vi "Main Page.vi"(8 "error in":errorcluster, 11 "Node Ptr":T2 format="%.0x") -> (0 "error out":errorcluster)   [LabVIEW 2020, in "Ballard ARINC 429 System Explorer.lvlib" / "Implementation.lvlib"]
uses:
  Implementation.lvlib
  <vilib>/NI VeriStand/Custom Device API/Custom Device API.lvlib
  Scripting/Ballard/Ballard ARINC 429 Scripting.lvlib
  Scripting/Ballard/Constants.vi
  <vilib>/NI VeriStand/Custom Device API/Custom Device Item Ref.ctl
  Shared/Initialization Method.ctl
panel:
  in  "Async Rx Execution":bool
  in  "General Header":cluster{"Section Name":string}={"Section Name"="Ballard ARINC 429 - Main"}
  in  "Initialization Method":T1
  in  "Core Number":i32=1 format="%o"
  in  "Number":i32=1 caption="PXI Slot Number"
  in  "SHDocVw.IWebBrowser":refnum<k7>(container)
  in  "Description":string
  in  "Name":string
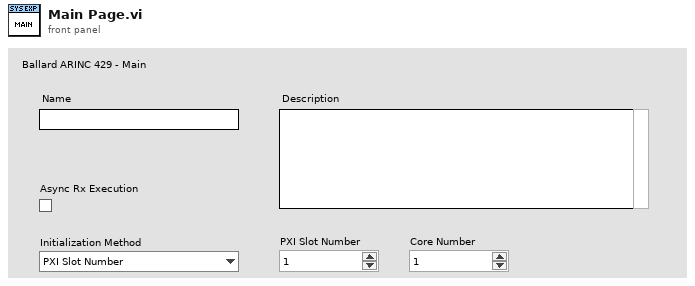
[diagram p1: front panel]
types:
  T1 = typedef "Initialization Method.ctl" = enum16{"PXI Slot Number", "Card Number", "Core Serial Number"}
  T2 = typedef "Custom Device API.lvlib/Custom Device Item Ref.ctl" = u64
  T3 = typedef "Device Parameters.ctl" = cluster{"initialization method":T1, "card number":i32, "PXI slot number":i32, "core number":i32, "core serial number":i32}
  T4 = typedef "Custom Device API.lvlib/Custom Device Item Info.ctl" = cluster{"Name":string, "Is Channel":bool, "GUID":string, "Is Waveform":bool}
  T5 = typedef "Custom Device API.lvlib/Custom Device Commands.ctl" = enum16{"Default", "Item renamed", "Shutdown", "Dynamic button pressed"}
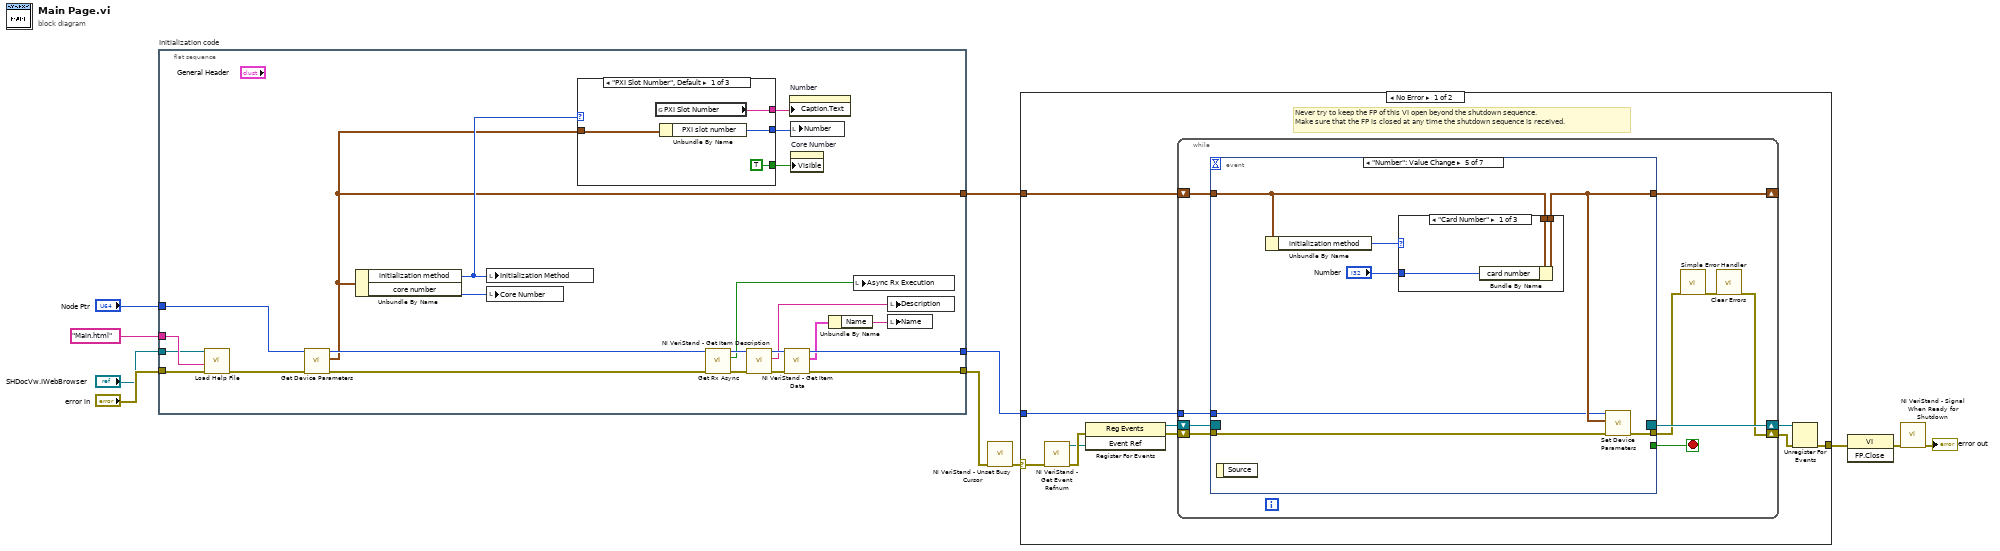
[diagram p0: block diagram]
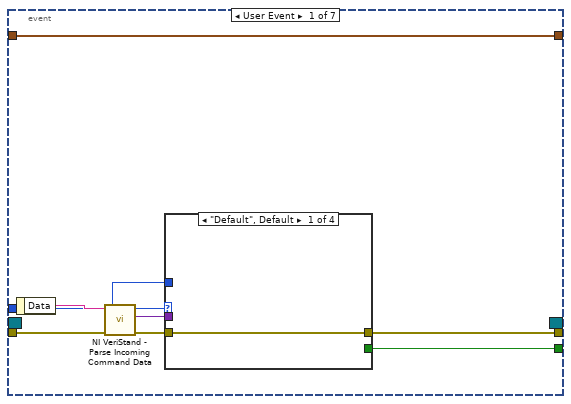
[diagram p2: hidden frame]
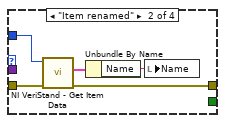
[diagram p3: hidden frame]
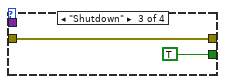
[diagram p4: hidden frame]
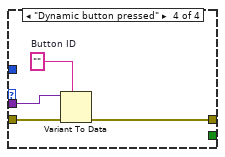
[diagram p5: hidden frame]
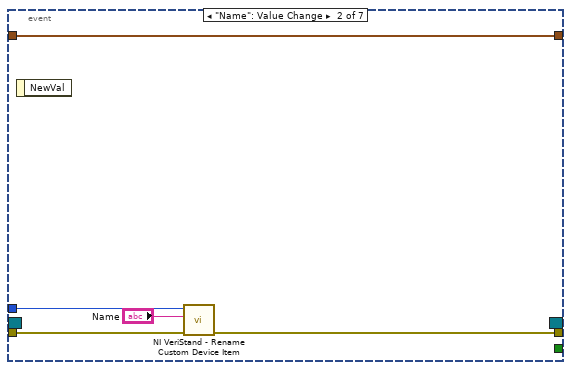
[diagram p6: hidden frame]
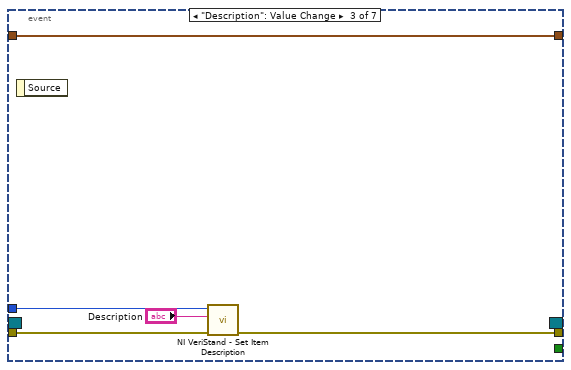
[diagram p7: hidden frame]
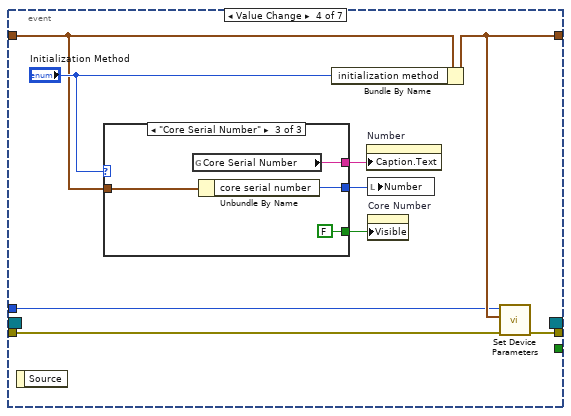
[diagram p8: hidden frame]
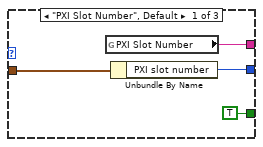
[diagram p9: hidden frame]
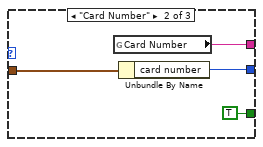
[diagram p10: hidden frame]
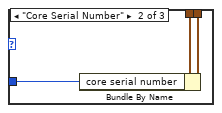
[diagram p11: hidden frame]
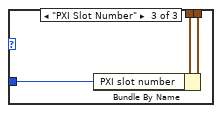
[diagram p12: hidden frame]
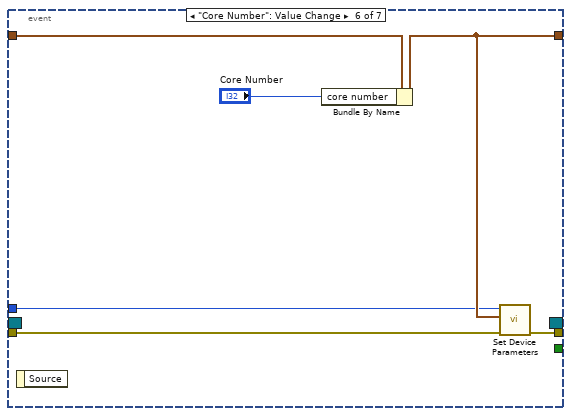
[diagram p13: hidden frame]
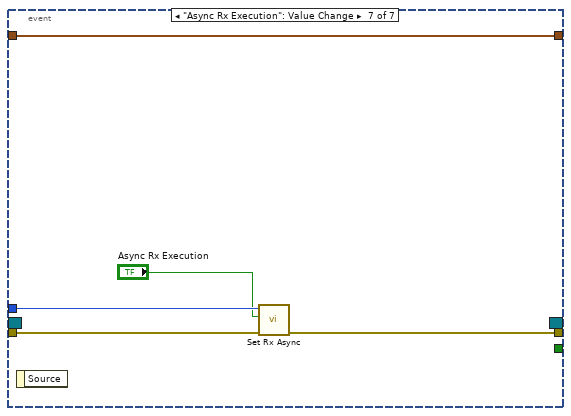
[diagram p14: hidden frame]
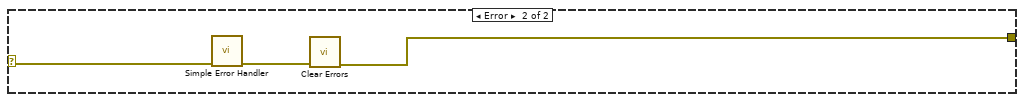
[diagram p15: hidden frame]
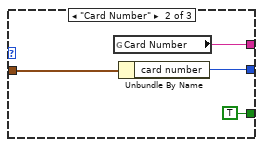
[diagram p16: hidden frame]
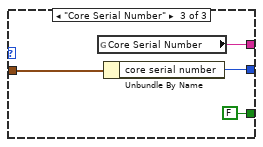
[diagram p17: hidden frame]
diagram:
  n1 = flat-sequence "Initialization code" {
    tunnel: "error in" -> [w27]
    tunnel: "Node Ptr" -> [w22]
    tunnel: [w30] -> w7
    tunnel: [w34] -> w4
    tunnel: "SHDocVw.IWebBrowser" -> [w25]
    tunnel: "Main.html" ("HTML File") -> [w26]
    tunnel: [w14] -> w1
    frame #0 {
      n2 = call "Load Help File.vi"("error in (no error)"=w27, "HTML File to Load"=w26, "Browser"=w25) -> ("error out"=w24:errorcluster)  [unwired: 8 in]
      n3 = call "Get Device Parameters.vi"("error in"=w24, "Ballard ARINC 429 custom device in"=w22) -> ("error out"=w18:errorcluster, "device parameters"=w14:T3, "Ballard ARINC 429 custom device out"=w23:T2)  [unwired: 7 in]
      n4 = Unbundle By Name(w14) -> ("initialization method"=w16:T1, "core number"=w21:i32)
      n5 = local write "Initialization Method"(w16) -> ()
      n6 = local write "Core Number"(w21) -> ()
      n7 = case shown="\"PXI Slot Number\", Default" w16 {
        tunnel: [w38 w42 w46] -> w15
        tunnel: w14 -> [w37 w41 w45]
        tunnel: [w36 w40 w44] -> w13
        tunnel: [TRUE ("Visible") TRUE ("Visible") FALSE ("Visible")] -> w12
        frame "PXI Slot Number", Default {
          n8 = global read "Constants.vi" "PXI Slot Number"() -> (w38:string)
          n9 = Unbundle By Name(w37) -> ("PXI slot number"=w36:i32)
        }
        frame "Card Number" {
          n10 = global read "Constants.vi" "Card Number"() -> (w42:string)
          n11 = Unbundle By Name(w41) -> ("card number"=w40:i32)
        }
        frame "Core Serial Number" {
          n12 = global read "Constants.vi" "Core Serial Number"() -> (w46:string)
          n13 = Unbundle By Name(w45) -> ("core serial number"=w44:i32)
        }
      }
      n14 = call "Get Rx Async.vi"("error in"=w18, "Ballard ARINC 429 custom device in"=w23) -> ("error out"=w19:errorcluster, "rx async?"=w17:bool, "Ballard ARINC 429 custom device out"=w20:T2)  [unwired: 7 in]
      n15 = call <vilib>:"NI VeriStand - Get Item Description.vi"("error in (no error)"=w19, "Item Ref in"=w20) -> ("error out"=w32:errorcluster, "Description"=w28:string, "Item Ref out"=w33:T2)  [unwired: 7 out]
      n16 = call <vilib>:"NI VeriStand - Get Item Data.vi"("error in (no error)"=w32, "Item Ref in"=w33) -> ("error out"=w30:errorcluster, "Item Info"=w31:T4, "Item Ref out"=w34:T2)  [unwired: 7 out]
      n17 = property on="Number" class="DigNum (strict)"("Caption.Text"=w15) -> ()  [unwired: 2 in, 2 out]
      n18 = local write "Number"(w13) -> ()
      n19 = property on="Core Number" class="DigNum (strict)"("Visible"=w12) -> ()  [unwired: 2 in, 2 out]
      n20 = Unbundle By Name(w31) -> ("Name"=w29:string)
      n21 = local write "Async Rx Execution"(w17) -> ()
      n22 = local write "Description"(w28) -> ()
      n23 = local write "Name"(w29) -> ()
    }
  }
  n24 = call <vilib>:"NI VeriStand - Unset Busy Cursor.vi"("error in (no error)"=w7) -> ("error out"=w6:errorcluster)  [unwired: 10 out]
  n25 = case shown="No Error" w6 {
    selector: w6 -> [w48 w148]
    tunnel: [w53 w146] -> w11
    tunnel: w4 -> [w49 _]
    tunnel: w1 -> [w47 _]
    frame No Error {
      # "Never try to keep the FP of this VI open beyond the shutdown sequence.\nMake sure that the FP is closed at any time the shutdown sequence is received."
      n26 = call <vilib>:"NI VeriStand - Get Event Refnum.vi"("error in (no error)"=w48) -> ("error out"=w56:errorcluster, "Event Ref"=w52:refnum<user-event>)  [unwired: 9 out]
      n27 = register-events(error in=w56, w52) -> (reference out=w50:refnum<event-registration>, error out=w51:errorcluster)  [unwired: 1 in]
      n28 = while {
        tunnel: w49 -> [w62]
        shift-right: [w59] -> w54
        shift-left: w51 -> [w65]
        shift-right: [w66] -> w55
        shift-left: w50 -> [w64]
        shift-right: [w57] -> _
        shift-left: w47 -> [w58]
        stop <- w63 stop-if-true
        n29 = event shown="[4] \"Number\": Value Change" {
          selector: w64 -> [_ _ _ _ _ _ _]
          dyn-events: [_ _ _ _ _ _ _] -> w66
          timeout: _ -> [_ _ _ _ _ _ _]
          tunnel: w65 -> [w75 w92 w96 w105 w123 w138 w144]
          tunnel: [w71 _ _ _ _ _ _] -> w63
          tunnel: [w70 w91 w95 w104 w122 w137 w141] -> w61
          tunnel: w62 -> [w69 w90 w97 w103 w120 w135 w143]
          tunnel: w58 -> [w67 w88 w93 w98 w125 w140 w145]
          tunnel: [w67 w88 w93 w106 w124 w139 w145] -> w57
          event User Event {
            n30 = event-data() -> ("Data"=w74:string)  [unwired: 1 out]
            n31 = call <vilib>:"NI VeriStand - Parse Incoming Command Data.vi"("error in (no error)"=w75, "Incoming data"=w74) -> ("error out"=w73:errorcluster, "Outgoing data"=w68:variant, "Action"=w72:T5)  [unwired: 7 out]
            n32 = case shown="\"Default\", Default" w72 {
              tunnel: w73 -> [w76 w81 w82 w87]
              tunnel: [_ _ TRUE _] -> w71
              tunnel: [w76 w78 w82 w84] -> w70
              tunnel: w69 -> [_ w80 _ _]
              tunnel: w68 -> [_ _ _ w86]
              frame "Default", Default {
              }
              frame "Item renamed" {
                n33 = call <vilib>:"NI VeriStand - Get Item Data.vi"("error in (no error)"=w81, "Item Ref in"=w80) -> ("error out"=w78:errorcluster, "Item Info"=w79:T4)  [unwired: 8 out]
                n34 = Unbundle By Name(w79) -> ("Name"=w77:string)
                n35 = local write "Name"(w77) -> ()
              }
              frame "Shutdown" {
              }
              frame "Dynamic button pressed" {
                w85 = ""  # Button ID
                n36 = Variant To Data(error in=w87, type=w85, Variant=w86) -> (error out=w84:errorcluster)  [unwired: 1 out]
              }
            }
          }
          event "Name": Value Change {
            n37 = event-data() -> ()  [unwired: 2 out]
            n38 = call <vilib>:"NI VeriStand - Rename Custom Device Item.vi"("error in (no error)"=w92, "New Name"="Name", "Item Ref in"=w90) -> ("error out"=w91:errorcluster)  [unwired: 1 in, 7 out]
          }
          event "Description": Value Change {
            n39 = event-data() -> ()  [unwired: 2 out]
            n40 = call <vilib>:"NI VeriStand - Set Item Description.vi"("error in (no error)"=w96, "Description"="Description", "Item Ref in"=w97) -> ("error out"=w95:errorcluster)  [unwired: 8 out]
          }
          event Value Change {
            n41 = event-data() -> ()  [unwired: 2 out]
            n42 = case shown="\"Core Serial Number\"" "Initialization Method" {
              tunnel: [w110 w114 w118] -> w102
              tunnel: w98 -> [w109 w113 w117]
              tunnel: [w108 w112 w116] -> w101
              tunnel: [TRUE ("Visible") TRUE ("Visible") FALSE ("Visible")] -> w100
              frame "PXI Slot Number", Default {
                n43 = global read "Constants.vi" "PXI Slot Number"() -> (w110:string)
                n44 = Unbundle By Name(w109) -> ("PXI slot number"=w108:i32)
              }
              frame "Card Number" {
                n45 = global read "Constants.vi" "Card Number"() -> (w114:string)
                n46 = Unbundle By Name(w113) -> ("card number"=w112:i32)
              }
              frame "Core Serial Number" {
                n47 = global read "Constants.vi" "Core Serial Number"() -> (w118:string)
                n48 = Unbundle By Name(w117) -> ("core serial number"=w116:i32)
              }
            }
            n49 = Bundle By Name(cluster=w98, "initialization method"="Initialization Method") -> (w106:T3)
            n50 = property on="Number" class="DigNum (strict)"("Caption.Text"=w102) -> ()  [unwired: 2 in, 2 out]
            n51 = local write "Number"(w101) -> ()
            n52 = property on="Core Number" class="DigNum (strict)"("Visible"=w100) -> ()  [unwired: 2 in, 2 out]
            n53 = call "Set Device Parameters.vi"("error in"=w105, "device parameters"=w106, "Ballard ARINC 429 custom device in"=w103) -> ("error out"=w104:errorcluster)  [unwired: 7 in, 1 out]
          }
          event "Number": Value Change {
            n54 = event-data() -> ()  [unwired: 2 out]
            n55 = Unbundle By Name(w125) -> ("initialization method"=w119:T1)
            n56 = case shown="\"Card Number\"" w119 {
              tunnel: w125 -> [w128 w131 w134]
              tunnel: [w127 w130 w133] -> w124
              tunnel: "Number" -> [w126 w129 w132]
              frame "Card Number" {
                n57 = Bundle By Name(cluster=w128, "card number"=w126) -> (w127:T3)
              }
              frame "Core Serial Number" {
                n58 = Bundle By Name(cluster=w131, "core serial number"=w129) -> (w130:T3)
              }
              frame "PXI Slot Number" {
                n59 = Bundle By Name(cluster=w134, "PXI slot number"=w132) -> (w133:T3)
              }
            }
            n60 = call "Set Device Parameters.vi"("error in"=w123, "device parameters"=w124, "Ballard ARINC 429 custom device in"=w120) -> ("error out"=w122:errorcluster)  [unwired: 7 in, 1 out]
          }
          event "Core Number": Value Change {
            n61 = event-data() -> ()  [unwired: 2 out]
            n62 = Bundle By Name(cluster=w140, "core number"="Core Number") -> (w139:T3)
            n63 = call "Set Device Parameters.vi"("error in"=w138, "device parameters"=w139, "Ballard ARINC 429 custom device in"=w135) -> ("error out"=w137:errorcluster)  [unwired: 7 in, 1 out]
          }
          event "Async Rx Execution": Value Change {
            n64 = event-data() -> ()  [unwired: 2 out]
            n65 = call "Set Rx Async.vi"("error in"=w144, "rx async?"="Async Rx Execution", "Ballard ARINC 429 custom device in"=w143) -> ("error out"=w141:errorcluster)  [unwired: 7 in, 1 out]
          }
        }
        n66 = call <vilib>:"Simple Error Handler.vi"("error in (no error)"=w61) -> ("error out"=w60:errorcluster)  [unwired: 1 in, 7 out]
        n67 = call <vilib>:"Clear Errors.vi"("error in (no error)"=w60) -> ("error out"=w59:errorcluster)  [unwired: 1 in, 5 out]
      }
      n68 = Unregister For Events(event registration refnum=w55, error in=w54) -> (error out=w53:errorcluster)
    }
    frame Error {
      n69 = call <vilib>:"Simple Error Handler.vi"("error in (no error)"=w148) -> ("error out"=w147:errorcluster)  [unwired: 1 in, 7 out]
      n70 = call <vilib>:"Clear Errors.vi"("error in (no error)"=w147) -> ("error out"=w146:errorcluster)  [unwired: 1 in, 5 out]
    }
  }
  n71 = invoke class="VI" method="FP.Close"(error in=w11) -> (error out=w10:errorcluster)  [unwired: 2 in, 2 out]
  n72 = call <vilib>:"NI VeriStand - Signal When Ready for Shutdown.vi"("error in (no error)"=w10) -> ("error out"=→"error out":errorcluster)  [unwired: 10 out]
